vi "loop_with_channel.vi"() -> ()   [LabVIEW 2021]
uses:
  <extravilib>/ChannelInstances/Stream-dbl/Read With Abort.vi
  <extravilib>/ChannelInstances/Stream-dbl/Write With Abort.vi
  <extravilib>/ChannelInstances/Stream-dbl/EndpointRead.vi
  <extravilib>/ChannelInstances/Stream-dbl/Endpoint.vi
  <extravilib>/ChannelInstances/Stream-dbl/Instantiate.vi
  <extravilib>/ChannelInstances/Stream-dbl/)Channel.vi
  <resource>/ChannelSupport/_ChannelSupport/WaitIfNeeded.vi
  <extravilib>/ChannelInstances/Stream-dbl.lvlib
panel:
  out "Waveform Chart 2":dbl[](graph)
  out "Waveform Chart":dbl(graph)
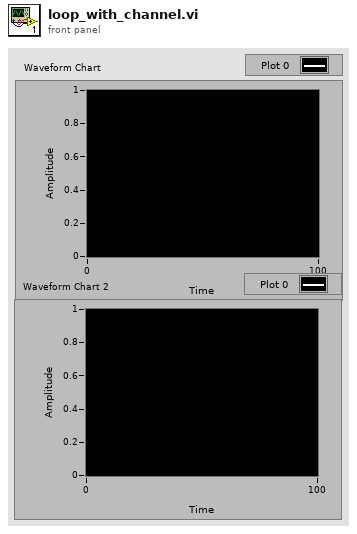
[diagram p1: front panel]
types:
  T1 = typedef "Stream-dbl.lvlib/)Channel.ctl" = refnum<queue>
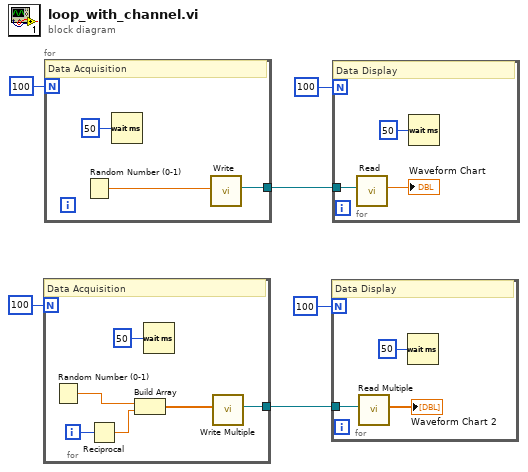
[diagram p0: block diagram]
diagram:
  n1 = for {
    N: 100 -> [_]
    tunnel: [w11] -> w1
    i -> [w8]
    # "Data Acquisition"
    n2 = Random Number (0-1)() -> (number: 0 to 1=w10:dbl)
    n3 = Reciprocal(x=w8) -> (1/x=w7:dbl)
    n4 = Build Array "Build Array"(w10, w7) -> (w9:dbl[])
    n5 = Wait (ms)(milliseconds to wait=u32 50) -> ()  [unwired: 1 out]
    n6 = call <extravilib>:"Write Multiple.vi"("elements"=w9) -> ("channel"=w11:T1)  [unwired: 7 in, 3 out]
  }
  n7 = for {
    N: 100 -> [_]
    tunnel: [w13] -> w4
    # "Data Acquisition"
    n8 = Random Number (0-1)() -> (number: 0 to 1=w14:dbl)
    n9 = Wait (ms)(milliseconds to wait=u32 50) -> ()  [unwired: 1 out]
    n10 = call <extravilib>:"Write.vi"("element"=w14) -> ("channel"=w13:T1)  [unwired: 8 in, 2 out]
  }
  n11 = for {
    N: 100 -> [_]
    tunnel: w1 -> [w17]
    # "Data Display"
    n12 = call <extravilib>:"Read Multiple.vi"("channel"=w17) -> ("elements"=→"Waveform Chart 2":dbl[])  [unwired: 7 in, 3 out]
    n13 = Wait (ms)(milliseconds to wait=u32 50) -> ()  [unwired: 1 out]
  }
  n14 = for {
    N: 100 -> [_]
    tunnel: w4 -> [w20]
    # "Data Display"
    n15 = call <extravilib>:"Read.vi"("channel"=w20) -> ("element"=→"Waveform Chart":dbl)  [unwired: 6 in, 4 out]
    n16 = Wait (ms)(milliseconds to wait=u32 50) -> ()  [unwired: 1 out]
  }
